vi "Read.vi"(5 "Username":string, 6 "Password":string, 7 "Address":string, 8 "Error In":errorcluster) -> (0 "Error Out":errorcluster)   [LabVIEW 2018, in "Tests.lvlib" / "SFTP File.lvlib"]
uses:
  SFTP File.lvlib
  src/Toolkit/SFTP File/Type Definitions/Open Options.ctl
  src/Toolkit/SFTP File/Support/Open from SFTP.vi
  src/Toolkit/SFTP File/Support/Close to SFTP.vi
  <vilib>/addons/_JKI Toolkits/Caraya/classes/Test/Test.lvclass
  <vilib>/addons/_JKI Toolkits/Caraya/classes/Assert/Assert.lvclass
  src/Toolkit/SFTP File/SFTP File.lvclass
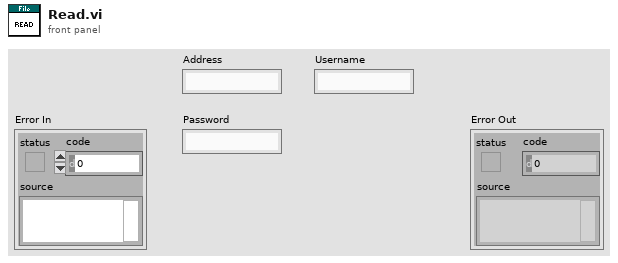
[diagram p1: front panel]
types:
  T1 = typedef "Toolkit.lvlib/SFTP File.lvclass/Open Options.ctl" = cluster{"Read":bool, "Write":bool, "Append":bool, "Create":bool, "Truncate":bool, "Exclude":bool}
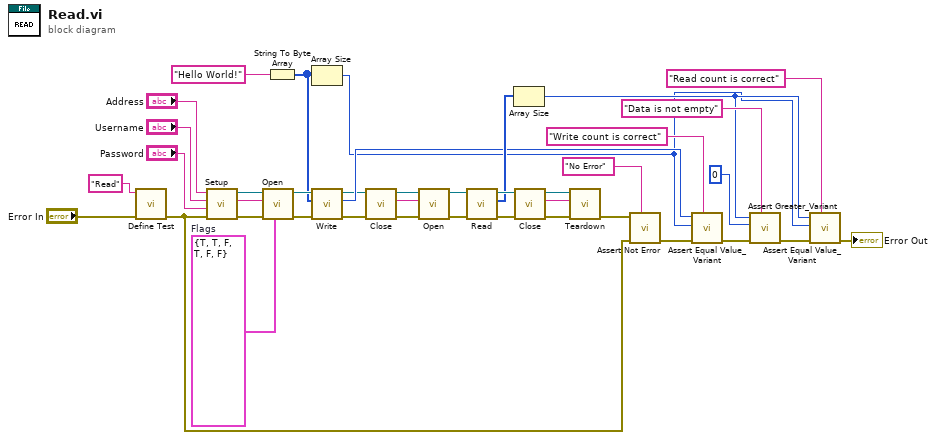
[diagram p0: block diagram]
diagram:
  w24 = T1 {"Read"=TRUE, "Write"=TRUE, "Append"=FALSE, "Create"=TRUE, "Truncate"=FALSE, "Exclude"=FALSE}  # Flags
  n1 = call <vilib>:"Define Test.vi"("error in (no error)"="Error In", "Label (VI Title)"="Read") -> ("error out"=w28:errorcluster)  [unwired: 9 in]
  n2 = call "Setup.vi"("Error In"=w28, "Password"="Password", "Username"="Username", "Address"="Address") -> ("Error Out"=w25:errorcluster, "Temporary File"=w2:string, "SFTP"=w26:refnum<class "SFTP.lvclass">)  [unwired: 5 in]
  n3 = call-poly "Open.vi"("Options"=w24, "Error In"=w25, "Remote Path"=w2, "SFTP"=w26) -> ("Error Out"=w22:errorcluster, "SFTP File"=w23:refnum<class "SFTP File.lvclass">)  [unwired: 6 in]
  n4 = String To Byte Array(string="Hello World!") -> (unsigned byte array=w20:u8[])
  n5 = Array Size(array=w20) -> (size(s)=w4:i32)
  n6 = call "Write.vi"("Error In"=w22, "Data"=w20, "SFTP File In"=w23) -> ("Error Out"=w14:errorcluster, "Count"=w17:i64, "SFTP File Out"=w15:refnum<class "SFTP File.lvclass">)  [unwired: 6 in]
  n7 = call-poly "Close.vi"("Error In"=w14, "SFTP File"=w15) -> ("Error Out"=w13:errorcluster, "Remote Path"=w1:string, "SFTP"=w12:refnum<class "SFTP.lvclass">)  [unwired: 7 in]
  n8 = call-poly "Open.vi"("Error In"=w13, "Remote Path"=w1, "SFTP"=w12) -> ("Error Out"=w11:errorcluster, "SFTP File"=w10:refnum<class "SFTP File.lvclass">)  [unwired: 7 in]
  n9 = call "Read.vi"("Error In"=w11, "SFTP File In"=w10) -> ("Error Out"=w36:errorcluster, "Data"=w35:u8[], "SFTP File Out"=w37:refnum<class "SFTP File.lvclass">)  [unwired: 7 in]
  n10 = Array Size(array=w35) -> (size(s)=w5:i32)
  n11 = call-poly "Close.vi"("Error In"=w36, "SFTP File"=w37) -> ("Error Out"=w8:errorcluster, "Remote Path"=w3:string, "SFTP"=w9:refnum<class "SFTP.lvclass">)  [unwired: 7 in]
  n12 = call "Teardown.vi"("Error In"=w8, "Temporary File"=w3, "SFTP"=w9) -> ("Error Out"=w27:errorcluster)  [unwired: 8 in]
  n13 = call <vilib>:"Assert Not Error.vi"("Label"="No Error", "error in (no error)"=w28, "Not Error?"=w27) -> ("error out"=w19:errorcluster)  [unwired: 8 in]
  n14 = call <vilib>:"Assert Equal Value_Variant.vi"("Label"="Write count is correct", "error in (no error)"=w19, "Y"=w4, "X"=w17) -> ("error out"=w18:errorcluster)  [unwired: 7 in]
  n15 = call <vilib>:"Assert Greater_Variant.vi"("Label"="Data is not empty", "error in (no error)"=w18, "Y"=0 ("size(s)"), "X"=w5) -> ("error out"=w34:errorcluster)  [unwired: 7 in]
  n16 = call <vilib>:"Assert Equal Value_Variant.vi"("Label"="Read count is correct", "error in (no error)"=w34, "Y"=w4, "X"=w5) -> ("error out"=→"Error Out":errorcluster)  [unwired: 7 in]
